vi "MCLB_ItemIndex_Tests.vi"(11 "error in":errorcluster) -> (15 "error out":errorcluster)   [LabVIEW 2016, in "DronaTest.lvlib"]
uses:
  DronaTest.lvlib
  APIs/Stimulus/ControlValue/SetValueAuto.vi
  APIs/Stimulus/ControlValue/Controls/MC Listbox/SetValueByItemIndex.vi
  APIs/Assert/AssertControlValue/Equal.vi
  APIs/Get/GetControlRef/GetControlRefByPath.vi
  <vilib>/addons/_JKI Toolkits/Caraya/classes/Test/Test.lvclass
  Drona.lvlib
  <vilib>/SLL Toolkit/SLL Debug/SLL Debug.lvlib
  APIs/Assert/AssertControlValue/AssertControlValue.lvlib
  <vilib>/addons/_JKI Toolkits/Caraya/classes/Assert/Assert.lvclass
  APIs/Stimulus/ControlValue/Controls/MC Listbox/StimulusMCListbox.lvlib
  APIs/Get/GetControlRef/GetControlRef.lvlib
  APIs/Stimulus/ControlValue/ControlValue.lvlib
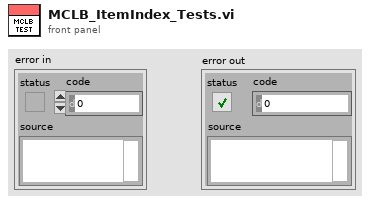
[diagram p1: front panel]
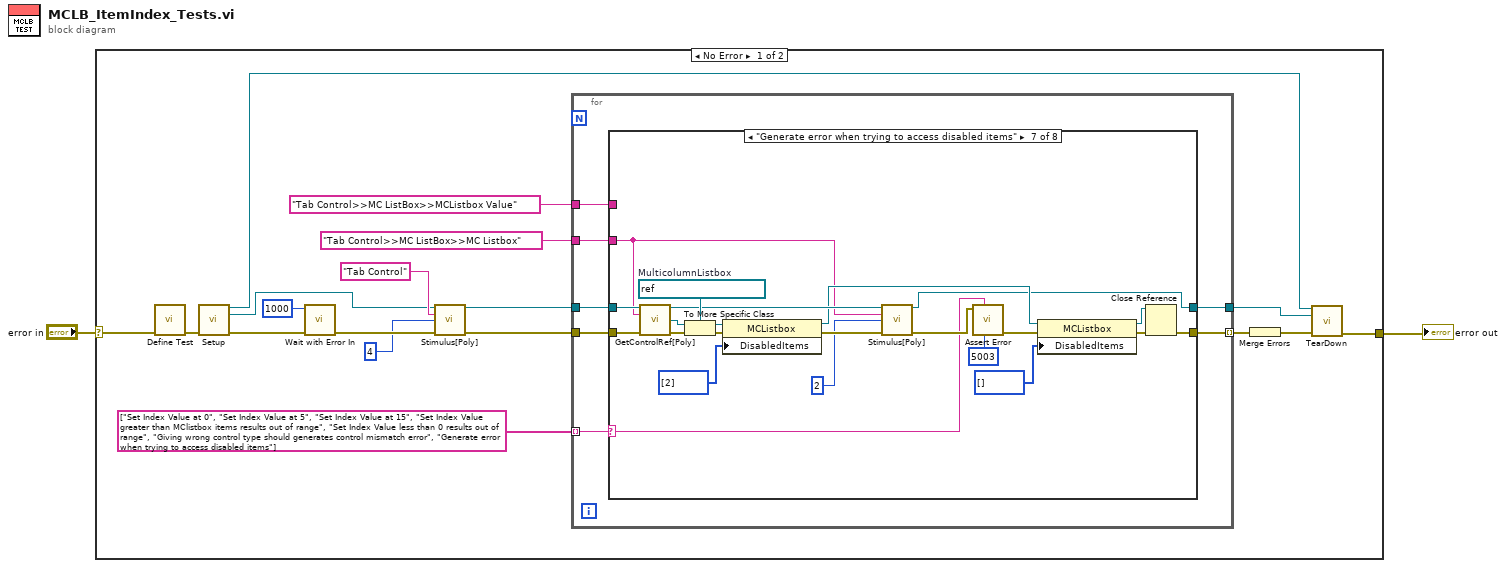
[diagram p0: block diagram]
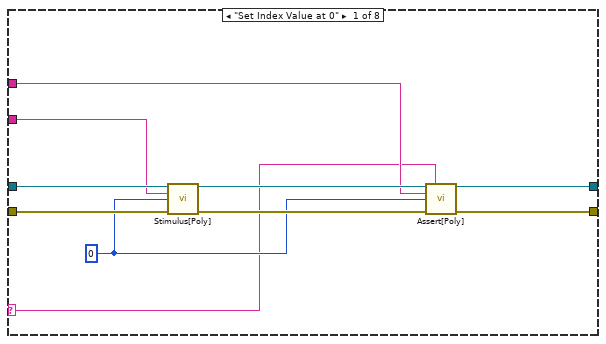
[diagram p2: hidden frame]
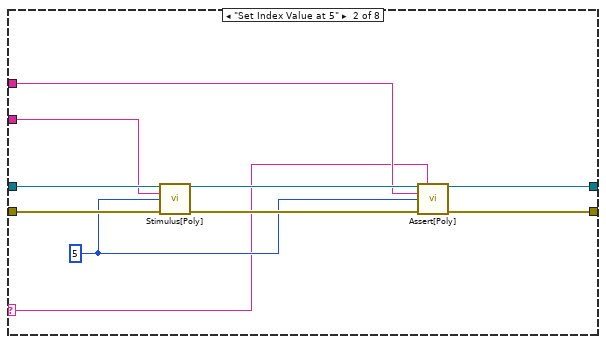
[diagram p3: hidden frame]
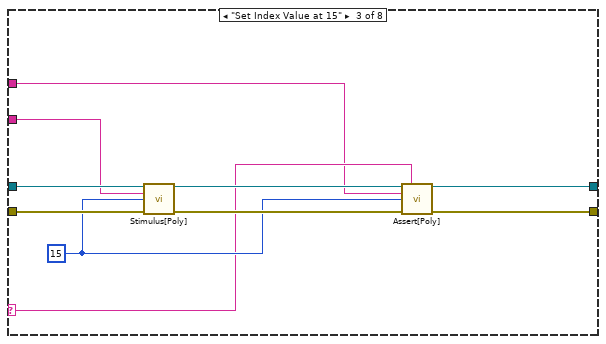
[diagram p4: hidden frame]
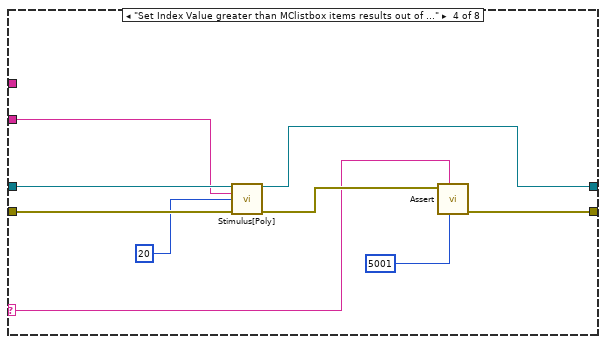
[diagram p5: hidden frame]
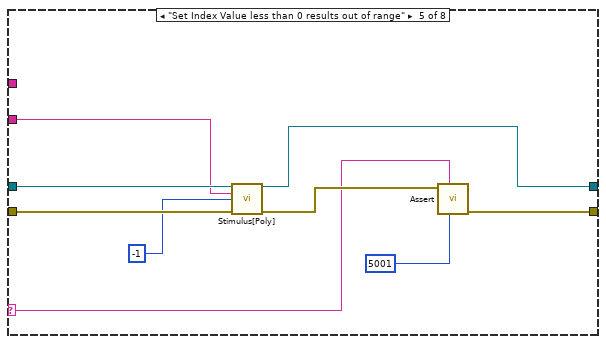
[diagram p6: hidden frame]
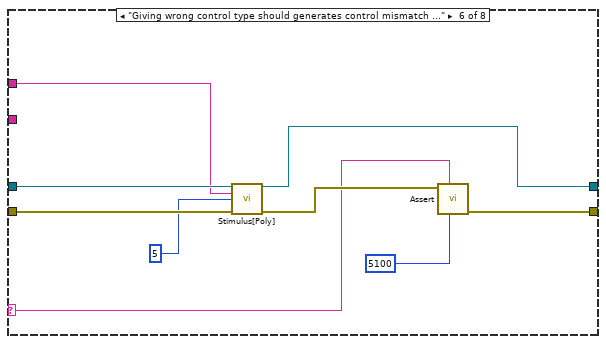
[diagram p7: hidden frame]
diagram:
  n1 = case shown="No Error" "error in" {
    selector: "error in" -> [w20 w109]
    tunnel: [w3 w109] -> w1
    frame No Error {
      n2 = call <vilib>:"Define Test.vi"("error in (no error)"=w20) -> ("error out"=w9:errorcluster)  [unwired: 9 in, 1 out]
      n3 = call "Setup.vi"("error in"=w9) -> ("Application Ref"=w5:refnum<vi>, "VI out"=w7:refnum<vi>, "error out"=w8:errorcluster)  [unwired: 12 in]
      n4 = call <vilib>:"Wait with Error In.vi"("error in (no error)"=w8, "milliseconds to wait"=u32 1000) -> ("error out"=w18:errorcluster)  [unwired: 9 in]
      n5 = call-poly "Stimulus[Poly].vi"("VI Reference In"=w7, "Control Path"="Tab Control", "Value (Signaling)"=4, "error in"=w18) -> ("VI Reference Out"=w14:refnum<vi>, "error out"=w17:errorcluster)  [unwired: 10 in]
      n6 = for {
        tunnel: w14 -> [w26]
        tunnel: "Tab Control>>MC ListBox>>MC Listbox" ("Control Path") -> [w25]
        tunnel: "Tab Control>>MC ListBox>>MCListbox Value" ("Control Path") -> [w24]
        tunnel: string[] ["Set Index Value at 0", "Set Index Value at 5", "Set Index Value at 15", "Set Index Value greater than MClistbox items results out of range", "Set Index Value less than 0 results out of range", "Giving wrong control type should generates control mismatch error", "Generate error when trying to access disabled items"] -> [w22] mode=indexing
        tunnel: [w21] -> w4
        tunnel: w17 -> [w27]
        tunnel: [w23] -> w10 mode=indexing
        n7 = case shown="\"Generate error when trying to access disabled items\"" w22 {
          selector: w22 -> [w28 w38 w50 w60 w69 w79 w87 _]
          tunnel: w27 -> [w37 w47 w57 w66 w75 w84 w106 w108]
          tunnel: w26 -> [w36 w46 w56 w65 w74 w83 w105 w107]
          tunnel: w25 -> [w32 w42 w48 w63 w72 _ w85 _]
          tunnel: w24 -> [w31 w41 w49 _ _ w76 _ _]
          tunnel: [w30 w40 w52 w61 w70 w80 w92 w108] -> w23
          tunnel: [w29 w39 w51 w58 w67 w77 w90 w107] -> w21
          frame "Set Index Value at 0" {
            w33 = 0 ("Item Index")
            n8 = call-poly "Stimulus[Poly].vi"("VI Reference In"=w36, "Control Path"=w32, "Item Index"=w33, "Error In"=w37) -> ("VI Reference Out"=w34:refnum<vi>, "Error Out"=w35:errorcluster)  [unwired: 10 in]
            n9 = call-poly "Assert[Poly].vi"("VI Reference In"=w34, "Test Label"=w28, "Control Path"=w31, "Control Value"=w33, "Error In"=w35) -> ("VI Reference Out"=w29:refnum<vi>, "Error Out"=w30:errorcluster)  [unwired: 8 in, 1 out]
          }
          frame "Set Index Value at 5" {
            w43 = 5 ("Item Index")
            n10 = call-poly "Stimulus[Poly].vi"("VI Reference In"=w46, "Control Path"=w42, "Item Index"=w43, "Error In"=w47) -> ("VI Reference Out"=w44:refnum<vi>, "Error Out"=w45:errorcluster)  [unwired: 10 in]
            n11 = call-poly "Assert[Poly].vi"("VI Reference In"=w44, "Test Label"=w38, "Control Path"=w41, "Control Value"=w43, "Error In"=w45) -> ("VI Reference Out"=w39:refnum<vi>, "Error Out"=w40:errorcluster)  [unwired: 8 in, 1 out]
          }
          frame "Set Index Value at 15" {
            w53 = 15 ("Item Index")
            n12 = call-poly "Stimulus[Poly].vi"("VI Reference In"=w56, "Control Path"=w48, "Item Index"=w53, "Error In"=w57) -> ("VI Reference Out"=w54:refnum<vi>, "Error Out"=w55:errorcluster)  [unwired: 10 in]
            n13 = call-poly "Assert[Poly].vi"("VI Reference In"=w54, "Test Label"=w50, "Control Path"=w49, "Control Value"=w53, "Error In"=w55) -> ("VI Reference Out"=w51:refnum<vi>, "Error Out"=w52:errorcluster)  [unwired: 8 in, 1 out]
          }
          frame "Set Index Value greater than MClistbox items results out of range" {
            n14 = call-poly "Stimulus[Poly].vi"("VI Reference In"=w65, "Control Path"=w63, "Item Index"=20, "Error In"=w66) -> ("VI Reference Out"=w58:refnum<vi>, "Error Out"=w62:errorcluster)  [unwired: 10 in]
            n15 = call-poly <vilib>:"Assert.vi"("error code (1)"=5001, "Label"=w60, "Error?"=w62) -> ("error out"=w61:errorcluster)  [unwired: 7 in, 1 out]
          }
          frame "Set Index Value less than 0 results out of range" {
            n16 = call-poly "Stimulus[Poly].vi"("VI Reference In"=w74, "Control Path"=w72, "Item Index"=-1, "Error In"=w75) -> ("VI Reference Out"=w67:refnum<vi>, "Error Out"=w71:errorcluster)  [unwired: 10 in]
            n17 = call-poly <vilib>:"Assert.vi"("error code (1)"=5001, "Label"=w69, "Error?"=w71) -> ("error out"=w70:errorcluster)  [unwired: 7 in, 1 out]
          }
          frame "Giving wrong control type should generates control mismatch error" {
            n18 = call-poly "Stimulus[Poly].vi"("VI Reference In"=w83, "Control Path"=w76, "Item Index"=5, "Error In"=w84) -> ("VI Reference Out"=w77:refnum<vi>, "Error Out"=w81:errorcluster)  [unwired: 10 in]
            n19 = call-poly <vilib>:"Assert.vi"("error code (1)"=5100, "Label"=w79, "Error?"=w81) -> ("error out"=w80:errorcluster)  [unwired: 7 in, 1 out]
          }
          frame "Generate error when trying to access disabled items" {
            w101 = refnum<vi> refnum  # MulticolumnListbox
            n20 = call-poly "GetControlRef[Poly].vi"("VI Reference In"=w105, "Control Path"=w85, "error In"=w106) -> ("VI Reference Out"=w97:refnum<vi>, "Ctl Refnum"=w102:refnum<vi>, "error out"=w104:errorcluster)  [unwired: 10 in]
            n21 = To More Specific Class(target class=w101, reference=w102, error in=w104) -> (specific class reference=w100:refnum<vi>, error out=w103:errorcluster)
            n22 = property class="MCListbox"(reference=w100, error in=w103, "DisabledItems"=i32[] [2] ("Disabled Items")) -> (reference out=w94:refnum<vi>, error out=w98:errorcluster)
            n23 = call-poly "Stimulus[Poly].vi"("VI Reference In"=w97, "Control Path"=w85, "Item Index"=2, "Error In"=w98) -> ("VI Reference Out"=w90:refnum<vi>, "Error Out"=w89:errorcluster)  [unwired: 10 in]
            n24 = call <vilib>:"Assert Error.vi"("error code (1)"=5003, "Label"=w87, "Error?"=w89) -> ("error out"=w88:errorcluster)  [unwired: 7 in, 1 out]
            n25 = property class="MCListbox"(reference=w94, error in=w88, "DisabledItems"=i32[] [] ("Disabled Items")) -> (reference out=w91:refnum<vi>, error out=w95:errorcluster)
            n26 = Close Reference(reference=w91, error in (no error)=w95) -> (error out=w92:errorcluster)
          }
          frame Default {
          }
        }
      }
      n27 = Merge Errors(w10) -> (w6:errorcluster)
      n28 = call "TearDown.vi"("Application Ref"=w5, "VI in"=w4, "error in (no error)"=w6) -> ("error out"=w3:errorcluster)  [unwired: 12 in]
    }
    frame Error {
    }
  }
  "error out" <- w1
